vi "set ACLR Tx Channel Offset.vi"(8 "error in (no error)":errorcluster, 10 "Tx Channel Offset (Hz)":dbl=1.0, 11 "FSV-40N in":refnum<class "FSV-40N.lvclass">) -> (0 "error out":errorcluster, 3 "FSV-40N out":refnum<class "FSV-40N.lvclass">)   [LabVIEW 2023, in "Spectrum Analyzer.lvlib" / "FSV-40N.lvclass"]
uses:
  FSV-40N.lvclass
  FSV-40N.lvclass/FSV-40N.ctl
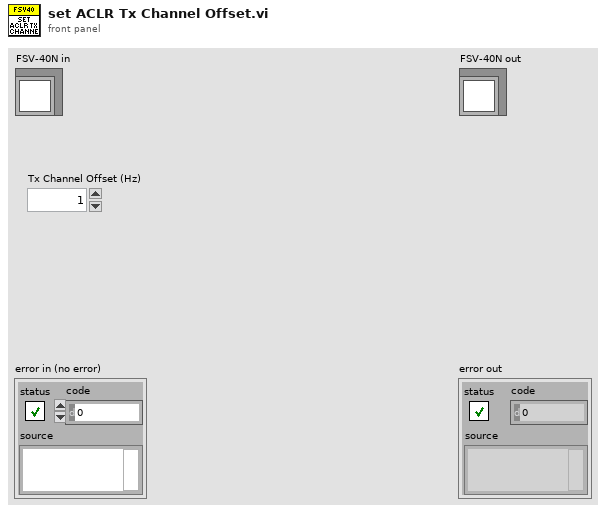
[diagram p1: front panel]
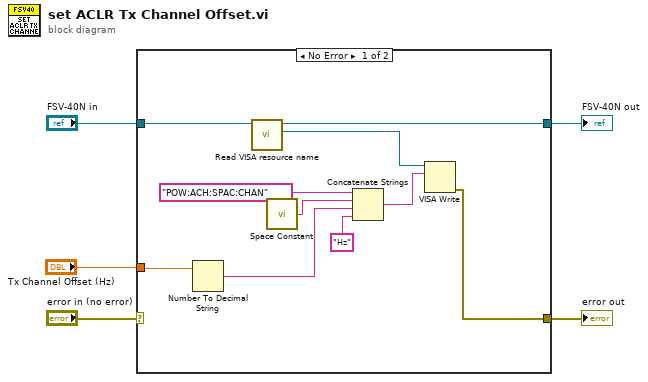
[diagram p0: block diagram]
diagram:
  n1 = case shown="No Error" "error in (no error)" {
    selector: "error in (no error)" -> [_ w16]
    tunnel: "FSV-40N in" -> [w15 w17]
    tunnel: [w8 w17] -> w3
    tunnel: [w7 w16] -> w2
    tunnel: "Tx Channel Offset (Hz)" -> [w12 _]
    frame No Error {
      n2 = Number To Decimal String(number=w12) -> (decimal integer string=w11:string)  [unwired: 1 in]
      n3 = call "Read VISA resource name.vi"("FSV-40N in"=w15) -> ("VISA resource name"=w10:refnum<visa-resource-name>, "FSV-40N out"=w8:refnum<class "FSV-40N.lvclass">)  [unwired: 8 in, 1 out]
      n4 = call <vilib>:"Space Constant.vi"() -> ("String"=w13:string)
      n5 = Concatenate Strings("POW:ACH:SPAC:CHAN" ("string"), w13, w11, "Hz" ("string")) -> (w9:string)
      n6 = VISA Write(VISA resource name=w10, write buffer=w9) -> (error out=w7:errorcluster)  [unwired: 1 in, 2 out]
    }
    frame Error {
    }
  }
  "error out" <- w2
  "FSV-40N out" <- w3
